vi "UsesDevOnly.vi"(0 "x":dbl) -> (4 "y":dbl)   [LabVIEW 2026, in "Lib.lvlib"]
doc: "Test fixture: calls DevDep.vi."
uses:
  Lib.lvlib
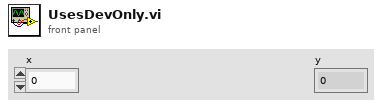
[diagram p1: front panel]
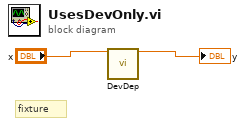
[diagram p0: block diagram]
diagram:
  # "fixture"
  n1 = call <vilib>:"DevDep.vi"("x"="x") -> ("y"=→"y":dbl)  [unwired: 14 in]
